vi "LABVIEW.vi"() -> ()   [LabVIEW 2015]
panel:
  in  "停止":bool
  out "波形图表":sgl(graph)
  out "temperature":sgl
  in  "sp":sgl
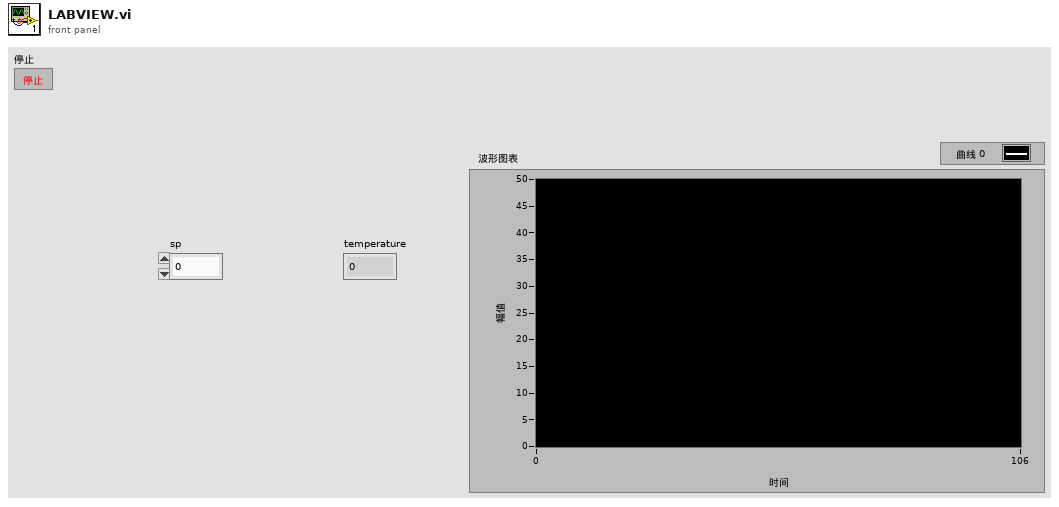
[diagram p1: front panel]
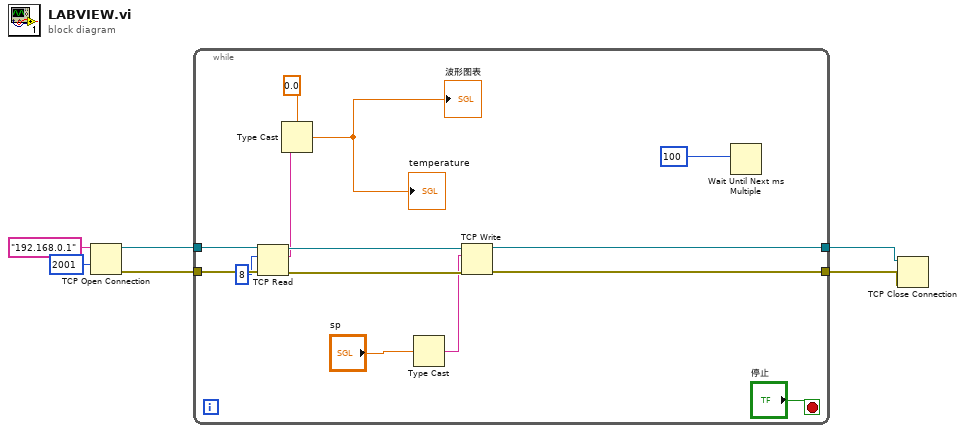
[diagram p0: block diagram]
diagram:
  n1 = TCP Open Connection(address="192.168.0.1" ("地址"), remote port or service name=u16 2001 ("远程端口或服务名称")) -> (connection ID=w1:refnum<k5>, error out=w3:errorcluster)  [unwired: 3 in]
  n2 = while {
    tunnel: [w18] -> w4
    tunnel: w3 -> [w17]
    tunnel: [w15] -> w2
    tunnel: w1 -> [w14]
    stop <- "停止" stop-if-true
    n3 = TCP Read(connection ID=w14, bytes to read=8 ("读取的字节"), error in (no error)=w17) -> (connection ID out=w19:refnum<k5>, data out=w11:string, error out=w16:errorcluster)  [unwired: 2 in]
    n4 = Type Cast(type=sgl 0.0, x=w11) -> (*(type *) &x=→"temperature" →"波形图表":sgl)
    n5 = Type Cast(x="sp") -> (*(type *) &x=w9:string)  [unwired: 1 in]
    n6 = TCP Write(connection ID=w19, data in=w9, error in (no error)=w16) -> (connection ID out=w18:refnum<k5>, error out=w15:errorcluster)  [unwired: 1 in, 1 out]
    n7 = Wait Until Next ms Multiple(millisecond multiple=u32 100 ("毫秒计时值")) -> ()  [unwired: 1 out]
  }
  n8 = TCP Close Connection(connection ID=w4, error in (no error)=w2) -> ()  [unwired: 1 in, 2 out]
